vi "global.vi"() -> (1 "dataset RID":string="dataset RID", 2 "API Key":string="nominal api key", 3 "command":string="config")   [LabVIEW 2020, in "Nominal-TDMS-Upload.lvlib" / "Nominal-TDMS-Upload.lvclass"]
uses:
  Nominal-TDMS-Upload.lvclass
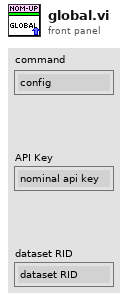
[diagram p1: front panel]
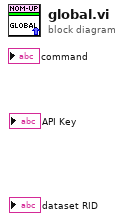
[diagram p0: block diagram]
diagram:
